vi "New Builder.vi"(8 "error in (no error)":errorcluster) -> (0 "error out":errorcluster, 3 "new reference":refnum<k24>)   [LabVIEW 2026, in "ToastNotification.lvlib" / "Toast Native.lvlib"]
doc: "Construct a native ToastContentBuilder. new reference is acquired by the caller, which must close it after its last use, including on partial initialization failure. Does not display a notification or register callbacks."
uses:
  Toast Native.lvlib
  C:/Users/loicw/Documents/LabVIEW/ToastNotifications/Sources/bins/Microsoft.Toolkit.Uwp.Notifications.dll
  bins/Microsoft.Toolkit.Uwp.Notifications.dll
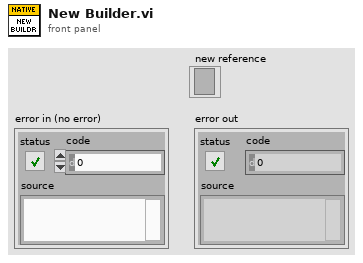
[diagram p1: front panel]
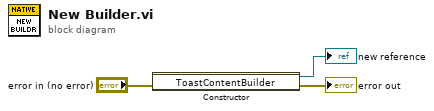
[diagram p0: block diagram]
diagram:
  n1 = constructor class="ToastContentBuilder"(error in="error in (no error)") -> (reference out=→"new reference":refnum<k24>, error out=→"error out":errorcluster)  [unwired: 2 in, 1 out]
